vi "Sort Indices by Key.vi"(8 "error in (no error)":errorcluster, 11 "Keys":dbl[](array[numeric])) -> (0 "error out":errorcluster, 3 "Sorted Indices":i32[](array[numeric]))   [LabVIEW 2024]
doc: "Returns the indices that put Keys in ascending order (a stable sort: equal keys keep their original order). Index the original array with each returned index to get it sorted. Used by the storage classes to sort rows by Sort Order or by Start Time.\n\nGenerated by: Claude"
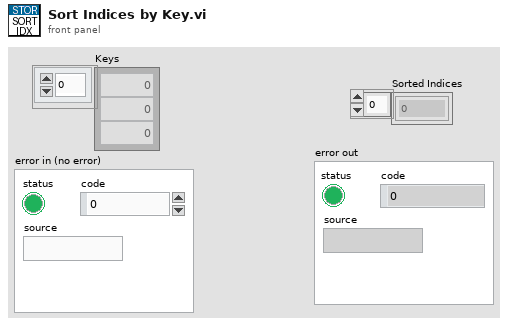
[diagram p1: front panel]
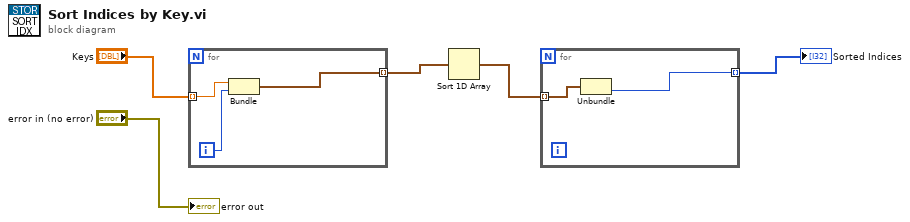
[diagram p0: block diagram]
diagram:
  n1 = for {
    tunnel: "Keys" -> [w7] mode=indexing
    tunnel: [w8] -> w3 mode=indexing
    i -> [w6]
    n2 = Bundle("Numeric"=w7, w6) -> (w8:cluster{"Numeric":dbl, i32})  [unwired: 1 in]
  }
  n3 = Sort 1D Array(array=w3) -> (sorted array=w4:cluster{"Numeric":dbl, i32}[])
  n4 = for {
    tunnel: w4 -> [w9] mode=indexing
    tunnel: [w10] -> w5 mode=indexing
    n5 = Unbundle(w9) -> (w10:i32)  [unwired: 1 out]
  }
  "Sorted Indices" <- w5
  "error out" <- "error in (no error)"
